vi "Board_Info_Ex.vi"() -> ()   [LabVIEW 2026]
uses:
  <vilib>/regexp/Match Regular Expression.xnode
panel:
  out "Neopixel":i32
  out "Servos":i32
  out "PWM Outputs":i32
  out "Analog Outputs":i32
  out "Analog Inputs":i32
  out "Digital Outputs":i32
  out "Digital Inputs":i32
  out "Tab Control":T1(tab)
  out "Placa":string
  out "Online":bool
  out "MAC":string
  out "Version":string
  out "Variant":string
  out "Valid Firmware":bool
  out "error out":errorcluster
  in  "VISA resource name":refnum<visa-resource-name>
  # "Board Info"
  # "Diagnostic"
  # "Outputs"
  # "Inputs"
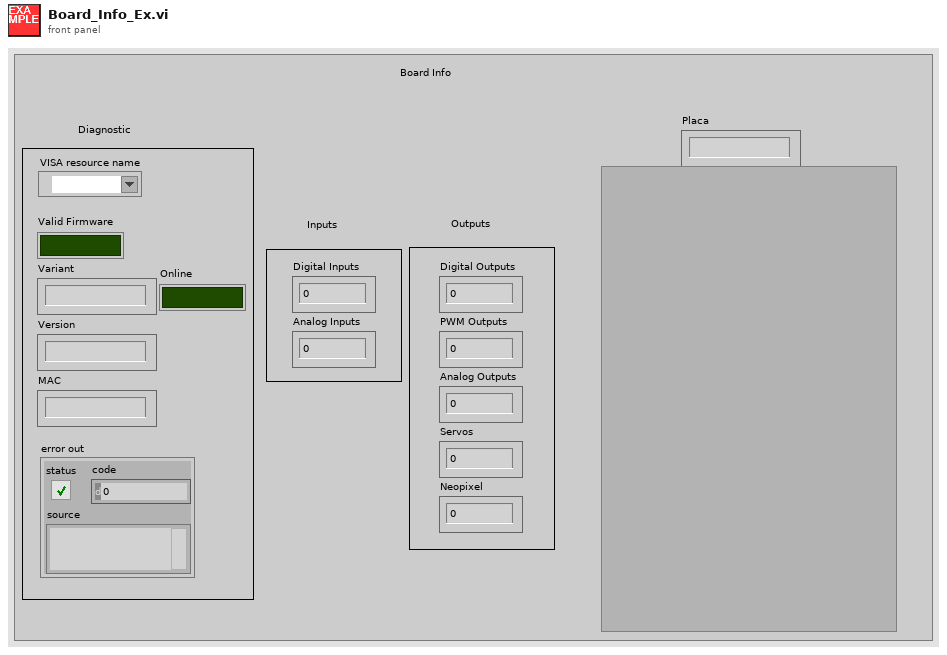
[diagram p1: front panel]
types:
  T1 = enum32{"IDLE", "ESP32", "NANO ESP32", "UNO", "NANO", "K8"}
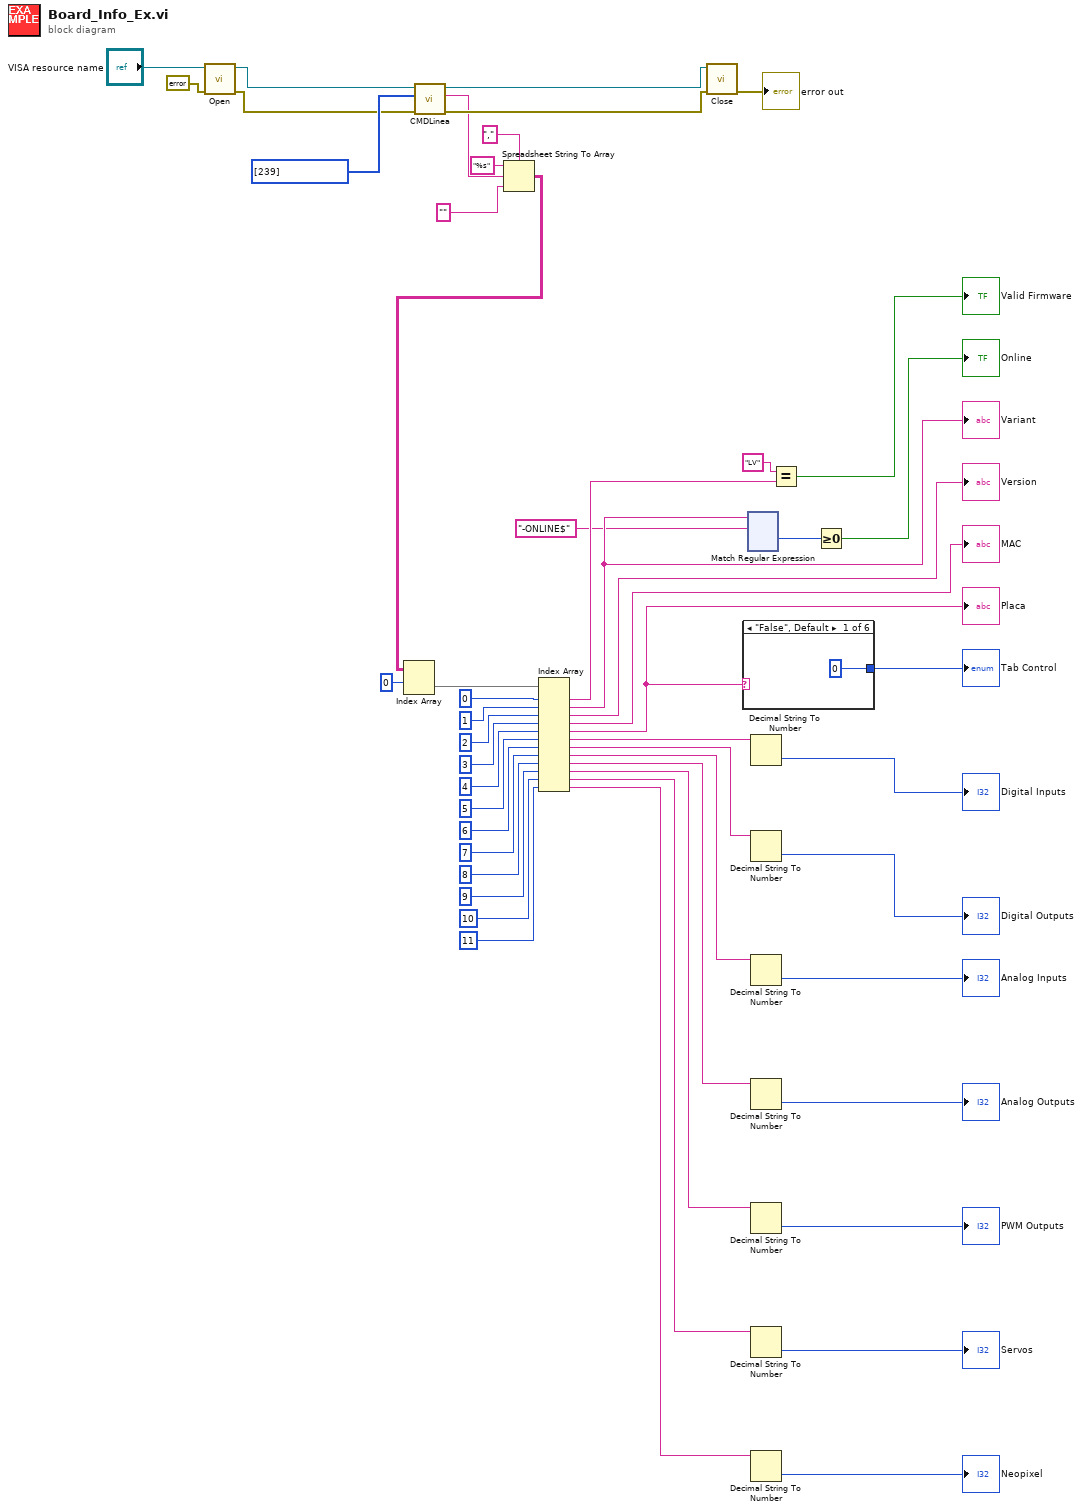
[diagram p0: block diagram]
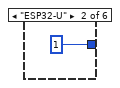
[diagram p2: hidden frame]
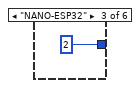
[diagram p3: hidden frame]
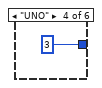
[diagram p4: hidden frame]
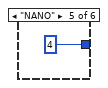
[diagram p5: hidden frame]
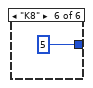
[diagram p6: hidden frame]
diagram:
  n1 = call "Open.vi"("error in (no error)"=errorcluster {"status"=FALSE, "code"=0, "source"=""}, "VISA resource name"="VISA resource name") -> ("error out"=w46:errorcluster, "VISA resource name out"=w49:refnum<visa-resource-name>)  [unwired: 8 in]
  n2 = call "CMDLinea.vi"("error in (no error)"=w46, "Comando"=u8[] [239], "VISA resource name"=w49) -> ("error out"=w45:errorcluster, "respuesta"=w44:string, "VISA resource name out"=w48:refnum<visa-resource-name>)  [unwired: 6 in]
  n3 = Spreadsheet String To Array(delimiter (Tab)=",", format string="%s", spreadsheet string=w44, array type (2D Dbl)="") -> (array=w40:string[][])
  n4 = Index Array(array=w40, index (row)=0) -> (element=w38:string[])  [unwired: 1 in]
  n5 = Index Array(array=w38, index #1=0 ("index"), index #2=1 ("index"), index #3=2 ("index"), index #4=3 ("index"), index #5=4 ("index"), index #6=5 ("index"), index #7=6 ("index"), index #8=7 ("index"), index #9=8 ("index"), index #10=9 ("index"), index #11=10 ("index"), index #12=11 ("index")) -> (element #1=w25:string, element #2=w22:string, element #3=→"Version":string, element #4=→"MAC":string, element #5=w16:string, element #6=w14:string, element #7=w13:string, element #8=w12:string, element #9=w11:string, element #10=w10:string, element #11=w9:string, element #12=w8:string)
  "Variant" <- w22
  "Placa" <- w16
  n6 = call "Close.vi"("error in (no error)"=w45, "VISA resource name"=w48) -> ("error out"=→"error out":errorcluster)  [unwired: 9 in]
  n7 = case shown="\"False\", Default" w16 {
    tunnel: [0 1 2 3 4 5] -> w15
    frame "False", Default {
    }
    frame "ESP32-U" {
    }
    frame "NANO-ESP32" {
    }
    frame "UNO" {
    }
    frame "NANO" {
    }
    frame "K8" {
    }
  }
  "Tab Control" <- w15
  n8 = xnode "Match Regular Expression"("input string"=w22, "regular expression"="-ONLINE$") -> ("offset past match"=w20:i32)  [unwired: 4 in, 4 out]
  n9 = Decimal String To Number(string=w14) -> (number=→"Digital Inputs":i32)  [unwired: 2 in, 1 out]
  n10 = Decimal String To Number(string=w13) -> (number=→"Digital Outputs":i32)  [unwired: 2 in, 1 out]
  n11 = Decimal String To Number(string=w12) -> (number=→"Analog Inputs":i32)  [unwired: 2 in, 1 out]
  n12 = Decimal String To Number(string=w11) -> (number=→"Analog Outputs":i32)  [unwired: 2 in, 1 out]
  n13 = Decimal String To Number(string=w10) -> (number=→"PWM Outputs":i32)  [unwired: 2 in, 1 out]
  n14 = Decimal String To Number(string=w9) -> (number=→"Servos":i32)  [unwired: 2 in, 1 out]
  n15 = Decimal String To Number(string=w8) -> (number=→"Neopixel":i32)  [unwired: 2 in, 1 out]
  n16 = Equal?(x="LV", y=w25) -> (x = y?=→"Valid Firmware":bool)
  n17 = Greater Or Equal To 0?(x=w20) -> (x >= 0?=→"Online":bool)
